vi "ShowUI.vi"(8 "error in":errorcluster, 9 "ShowUI":bool, 11 "UI_Library in":refnum<class "UI_Library.lvclass">) -> (0 "error out":errorcluster, 3 "UI_Library out":refnum<class "UI_Library.lvclass">)   [LabVIEW 2018, in "UI_Library.lvlib" / "UI_Library.lvclass"]
uses:
  UI_Library.lvclass
  UI_Library.lvclass/UI_Library.ctl
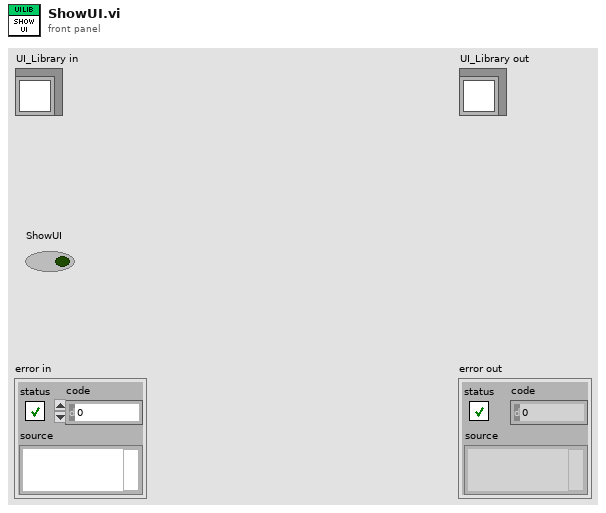
[diagram p1: front panel]
types:
  T1 = enum32{"Invalid", "Standard", "Closed", "Hidden", "Minimized", "Maximized"}
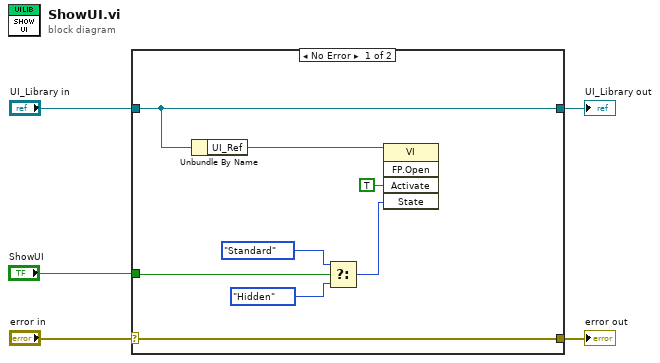
[diagram p0: block diagram]
diagram:
  n1 = case shown="No Error" "error in" {
    selector: "error in" -> [w13 w15]
    tunnel: [w13 w15] -> w4
    tunnel: [w12 w14] -> w2
    tunnel: "UI_Library in" -> [w12 w14]
    tunnel: "ShowUI" -> [w10 _]
    frame No Error {
      n2 = Unbundle By Name(w12) -> ("UI_Ref"=w11:refnum<vi>)
      n3 = Select(t=T1."Standard" ("State"), s=w10, f=T1."Hidden" ("State")) -> (s? t:f=w9:T1)
      n4 = invoke class="VI" method="FP.Open"(reference=w11, "Activate"=TRUE ("Activate?"), "State"=w9) -> ()  [unwired: 2 in, 5 out]
    }
    frame Error {
    }
  }
  "error out" <- w4
  "UI_Library out" <- w2
